vi "ADCS.UnlockECUSecurity.vi"(6 "Diagnostic Protocol":T3, 7 "Addon Name":string, 8 "error in (no error)":errorcluster, 9 "MasterKey":string, 10 "Security":T1={"Type"=enum."None", "Source DLL Path"=path "", "Target DLL Path"=path "", "Security Level"=1, "Static Master Key"="", "Max Key Length"=1, "Host IP Address"="", "ECU  Variant"=0, "Optional Parameter"=0}, 11 "diag ref in":T4={"Diag CAN Handle"=0, "Transport Protocol"=enum."ISO TP - Normal Mode", "Receive Address Extension"=0, "Transmit Address Extension"=0, "Receive CAN Id"=0, "Transmit CAN Id"=0, "Log Frames ?"=FALSE, "My TP Address"=0, "Other TP Address"=0, "T1"=0, "T2"=0, "T3"=0, "T4"=0, "Tx SN"=0, "Block Size"=0, "Rx SN"=0, "VW TP Initialized?"=FALSE, "Tx block no"=0, "baud rate"=0, "Interface"="", "Channel Diag CAN Handle"=0, "UDP Connection ID"=refnum, "TCP Connection ID"=refnum, "Target IP Addr"=0, "Source Address"=0, "Target Address"=0, "Send Header NACK?"=FALSE, "DLL Handle"=0, "NAD"=0, "Time Stamp read first"=0.0, "Time Stamp read last"=0.0, "Time Stamp write first"=0.0, "Time Stamp write last"=0.0, "Time Stamp write"=0.0, "Time Stamp read"=0.0, " I/O Mode"=0, "FD Baudrate"=0, "TX_DL"=8, "RX_DL"=8, "DoIP Protocol Version"=1, " Selected I/O Mode"=0, "TesterPresent Counter"=0, "TesterPresent Limit"=0, "TesterPresent Tick[ms]"=10, "TesterPresent RequireResponse?"=FALSE, "TesterPresent Stored Ref?"=FALSE, "TesterPresent Message"=[], "TesterPresent Task Handle"=0, "TesterPresent Semaphore"=refnum, "Response Plausibility Check"=1, "Default Version?"=TRUE, "Diagostic Globals"={"Timeout FC (Bs)"=250, "Timeout CF (Cr)"=250, "Timeout Diag Command"=1000, "Receive Block Size (BS)"=0, "Wait Time CF (STmin)"=5, "Max Waits (N_WFTmax)"=10, "Waits to Send (N_WAIT)"=0, "Time between Waits (TW)"=25, "Fill CAN Frames?"=TRUE, "Fill Byte"=255, "Invalid Response as Error?"=FALSE, "Max RspPending Count"=5, "VWTP Command Timeout"=50, "Transport Protocol"=enum."Diagnostics on IP", "Diag CAN Handle"=0, "DLL Handle"=0, "Timeout RspPending"=1000}, "Session-based Properties?"=FALSE, "NI-XNET IP Stack Reference"=0, "NI-XNET IP Stack TCP Reference"=-1, "NI-XNET IP Stack UDP Reference"=-1, "NI-XNET IP Stack Local Interface"="", "Functional CAN Id"=0, "Diag CAN Queue"=refnum, "Frame Fillling Mode"=0, "DoIP Acknowledge Mode"=0, "Message Buffer"=[]} {"Diagostic Globals"."Fill Byte" format="%x"; "TesterPresent Message" format="%.0x"; "Selected I/O Mode" items=["CAN", "CAN FD", "CAN FD+BRS", "ECU Determined"]; "DoIP Protocol Version" items=["2010"=1, "2012"=2]; "RX_DL" items=["8"=8, "12"=12, "16"=16, "20"=20, "24"=24, "32"=32, "48"=48, "64"=64]; "TX_DL" items=["8"=8, "12"=12, "16"=16, "20"=20, "24"=24, "32"=32, "48"=48, "64"=64]; "I/O Mode" items=["CAN", "CAN FD", "CAN FD+BRS", "Not yet determined"]}) -> (0 "error out":errorcluster, 1 "success?":bool, 3 "diag ref out":T4={"Diag CAN Handle"=0, "Transport Protocol"=enum."ISO TP - Normal Mode", "Receive Address Extension"=0, "Transmit Address Extension"=0, "Receive CAN Id"=0, "Transmit CAN Id"=0, "Log Frames ?"=FALSE, "My TP Address"=0, "Other TP Address"=0, "T1"=0, "T2"=0, "T3"=0, "T4"=0, "Tx SN"=0, "Block Size"=0, "Rx SN"=0, "VW TP Initialized?"=FALSE, "Tx block no"=0, "baud rate"=0, "Interface"="", "Channel Diag CAN Handle"=0, "UDP Connection ID"=refnum, "TCP Connection ID"=refnum, "Target IP Addr"=0, "Source Address"=0, "Target Address"=0, "Send Header NACK?"=FALSE, "DLL Handle"=0, "NAD"=0, "Time Stamp read first"=0.0, "Time Stamp read last"=0.0, "Time Stamp write first"=0.0, "Time Stamp write last"=0.0, "Time Stamp write"=0.0, "Time Stamp read"=0.0, " I/O Mode"=0, "FD Baudrate"=0, "TX_DL"=8, "RX_DL"=8, "DoIP Protocol Version"=1, " Selected I/O Mode"=0, "TesterPresent Counter"=0, "TesterPresent Limit"=0, "TesterPresent Tick[ms]"=10, "TesterPresent RequireResponse?"=FALSE, "TesterPresent Stored Ref?"=FALSE, "TesterPresent Message"=[], "TesterPresent Task Handle"=0, "TesterPresent Semaphore"=refnum, "Response Plausibility Check"=1, "Default Version?"=TRUE, "Diagostic Globals"={"Timeout FC (Bs)"=250, "Timeout CF (Cr)"=250, "Timeout Diag Command"=1000, "Receive Block Size (BS)"=0, "Wait Time CF (STmin)"=5, "Max Waits (N_WFTmax)"=10, "Waits to Send (N_WAIT)"=0, "Time between Waits (TW)"=25, "Fill CAN Frames?"=TRUE, "Fill Byte"=255, "Invalid Response as Error?"=FALSE, "Max RspPending Count"=5, "VWTP Command Timeout"=50, "Transport Protocol"=enum."Diagnostics on IP", "Diag CAN Handle"=0, "DLL Handle"=0, "Timeout RspPending"=1000}, "Session-based Properties?"=FALSE, "NI-XNET IP Stack Reference"=0, "NI-XNET IP Stack TCP Reference"=-1, "NI-XNET IP Stack UDP Reference"=-1, "NI-XNET IP Stack Local Interface"="", "Functional CAN Id"=0, "Diag CAN Queue"=refnum, "Frame Fillling Mode"=0, "DoIP Acknowledge Mode"=0, "Message Buffer"=[]} {"Diagostic Globals"."Fill Byte" format="%x"; "TesterPresent Message" format="%.0x"; "Selected I/O Mode" items=["CAN", "CAN FD", "CAN FD+BRS", "ECU Determined"]; "DoIP Protocol Version" items=["2010"=1, "2012"=2]; "RX_DL" items=["8"=8, "12"=12, "16"=16, "20"=20, "24"=24, "32"=32, "48"=48, "64"=64]; "TX_DL" items=["8"=8, "12"=12, "16"=16, "20"=20, "24"=24, "32"=32, "48"=48, "64"=64]; "I/O Mode" items=["CAN", "CAN FD", "CAN FD+BRS", "Not yet determined"]})   [LabVIEW 2024, in "Diagnostics Addon Engine.lvlib"]
uses:
  Diagnostics Addon Engine.lvlib
  <vilib>/Automotive Diagnostic Command Set/Diagnostic Transport.llb/Diag Reference.ctl
  <vilib>/Automotive Diagnostic Command Set/Diagnostic Transport.llb/Transport Protocol Selector.ctl
  <vilib>/Automotive Diagnostic Command Set/Diagnostic Transport.llb/DoIP Protocol Version.ctl
  <vilib>/Automotive Diagnostic Command Set/Diagnostic Transport.llb/Diag Globals.ctl
  Addon Shared/Types/Protocol.ctl
  Addon Shared/Types/Security.ctl
  Addon Shared/Types/Security.Type.ctl
  <vilib>/NI/STM/TCP/TCP Read Options.ctl
  <vilib>/NI/STM/TCP/Get Connection Reference (TCP).vi
  Support Libraries/GMLAN/_SubVIs/SecurityAccess_sendKey.vi
  <vilib>/NI/STM/TCP/Read Meta Data (TCP Ref).vi
  Support Libraries/GMLAN/_SubVIs/SecurityAccess_requestSeed.vi
  <vilib>/NI/STM/TCP/Read Meta Data (TCP Clst).vi
  <vilib>/Automotive Diagnostic Command Set/Diagnostic Transport.llb/Diagnostic Service.vi
  <vilib>/Automotive Diagnostic Command Set/Diagnostic Transport.llb/Apply Success Failure Error.vi
  <vilib>/Utility/error.llb/Error Cluster From Error Code.vi
  Support Libraries/GMLAN/GMLAN.lvlib
  <vilib>/NI/STM/NI STM.lvlib
  <vilib>/NI/NI VeriStand Addon Network Comm/Shared/NI VeriStand Addon Network Comm Shared.lvlib
  <vilib>/addons/Automotive Diagnostic Command Set/NI_Automotive Diagnostic Command Set.lvlib
  Addon Shared/Diagnostics Addon Shared.lvlib
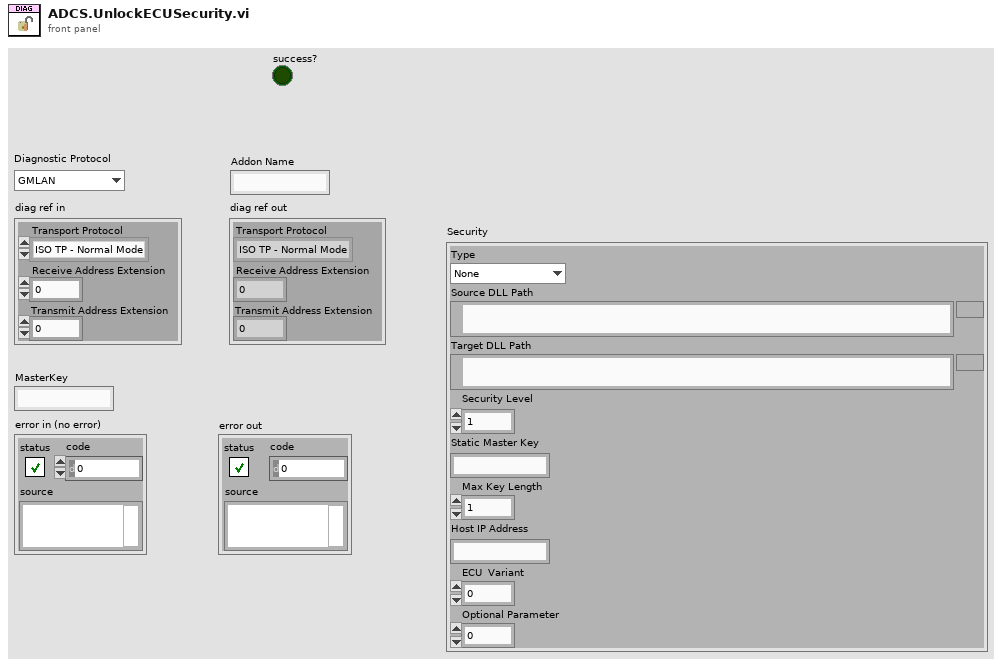
[diagram p1: front panel]
types:
  T1 = typedef "Diagnostics Addon Shared.lvlib/Security.ctl" = cluster{"Type":T2, "Source DLL Path":path, "Target DLL Path":path, "Security Level":u32, "Static Master Key":string, "Max Key Length":u32, "Host IP Address":string, "ECU  Variant":i8, "Optional Parameter":i8}
  T2 = typedef "Diagnostics Addon Shared.lvlib/Security.Type.ctl" = enum16{"None", "SeedKey DLL", "MasterKey (Channel)", "MasterKey (Static)", "SeedKey DLL (Windows)"}
  T3 = typedef "Diagnostics Addon Shared.lvlib/Protocol.ctl" = enum16{"GMLAN", "KWP-2000", "UDS", "User-Defined"}
  T4 = typedef "NI_Automotive Diagnostic Command Set.lvlib/Diag Reference.ctl" = cluster{"Diag CAN Handle":u32, "Transport Protocol":T5, "Receive Address Extension":u8, "Transmit Address Extension":u8, "Receive CAN Id":u32, "Transmit CAN Id":u32, "Log Frames ?":bool, "My TP Address":u8, "Other TP Address":u8, "T1":u16, "T2":u16, "T3":u16, "T4":u16, "Tx SN":u8, "Block Size":u8, "Rx SN":u8, "VW TP Initialized?":bool, "Tx block no":u8, "baud rate":u64, "Interface":string, "Channel Diag CAN Handle":u32, "UDP Connection ID":refnum<k16>, "TCP Connection ID":refnum<k5>, "Target IP Addr":u32, "Source Address":u16, "Target Address":u16, "Send Header NACK?":bool, "DLL Handle":u32, "NAD":u8, "Time Stamp read first":dbl, "Time Stamp read last":dbl, "Time Stamp write first":dbl, "Time Stamp write last":dbl, "Time Stamp write":dbl, "Time Stamp read":dbl, " I/O Mode":u32, "FD Baudrate":u64, "TX_DL":u16, "RX_DL":u16, "DoIP Protocol Version":T6, " Selected I/O Mode":u32, "TesterPresent Counter":u32, "TesterPresent Limit":u32, "TesterPresent Tick[ms]":i32, "TesterPresent RequireResponse?":bool, "TesterPresent Stored Ref?":bool, "TesterPresent Message":u8[], "TesterPresent Task Handle":i32, "TesterPresent Semaphore":T7, "Response Plausibility Check":u32, "Default Version?":bool, "Diagostic Globals":T8, "Session-based Properties?":bool, "NI-XNET IP Stack Reference":i64, "NI-XNET IP Stack TCP Reference":i64, "NI-XNET IP Stack UDP Reference":i64, "NI-XNET IP Stack Local Interface":string, "Functional CAN Id":u32, "Diag CAN Queue":refnum<queue>, "Frame Fillling Mode":u32, "DoIP Acknowledge Mode":u32, "Message Buffer":u8[]}
  T5 = typedef "NI_Automotive Diagnostic Command Set.lvlib/Transport Protocol Selector.ctl" = enum16{"ISO TP - Normal Mode", "ISO TP - Mixed Mode", "VW TP 2.0", "Diagnostics on IP", "ISO TP LIN"}
  T6 = typedef "NI_Automotive Diagnostic Command Set.lvlib/DoIP Protocol Version.ctl" = u8
  T7 = typedef "Semaphore RefNum" = refnum<k1>
  T8 = typedef "NI_Automotive Diagnostic Command Set.lvlib/Diag Globals.ctl" = cluster{"Timeout FC (Bs)":u32, "Timeout CF (Cr)":u32, "Timeout Diag Command":u32, "Receive Block Size (BS)":u8, "Wait Time CF (STmin)":u8, "Max Waits (N_WFTmax)":u8, "Waits to Send (N_WAIT)":i32, "Time between Waits (TW)":u32, "Fill CAN Frames?":bool, "Fill Byte":u32, "Invalid Response as Error?":bool, "Max RspPending Count":u32, "VWTP Command Timeout":u32, "Transport Protocol":T5, "Diag CAN Handle":u32, "DLL Handle":u32, "Timeout RspPending":u32}
  T9 = typedef "NI STM.lvlib/TCP Read Options.ctl" = cluster{"ignore timeout error":bool, "timeout ms (1000)":i32}
  T10 = typedef "NI STM.lvlib/TCP Connection Info.ctl" = cluster{"connection ID":refnum<k5>, "meta data":T11[]}
  T11 = typedef "NI STM.lvlib/MetaDataElement.ctl" = string
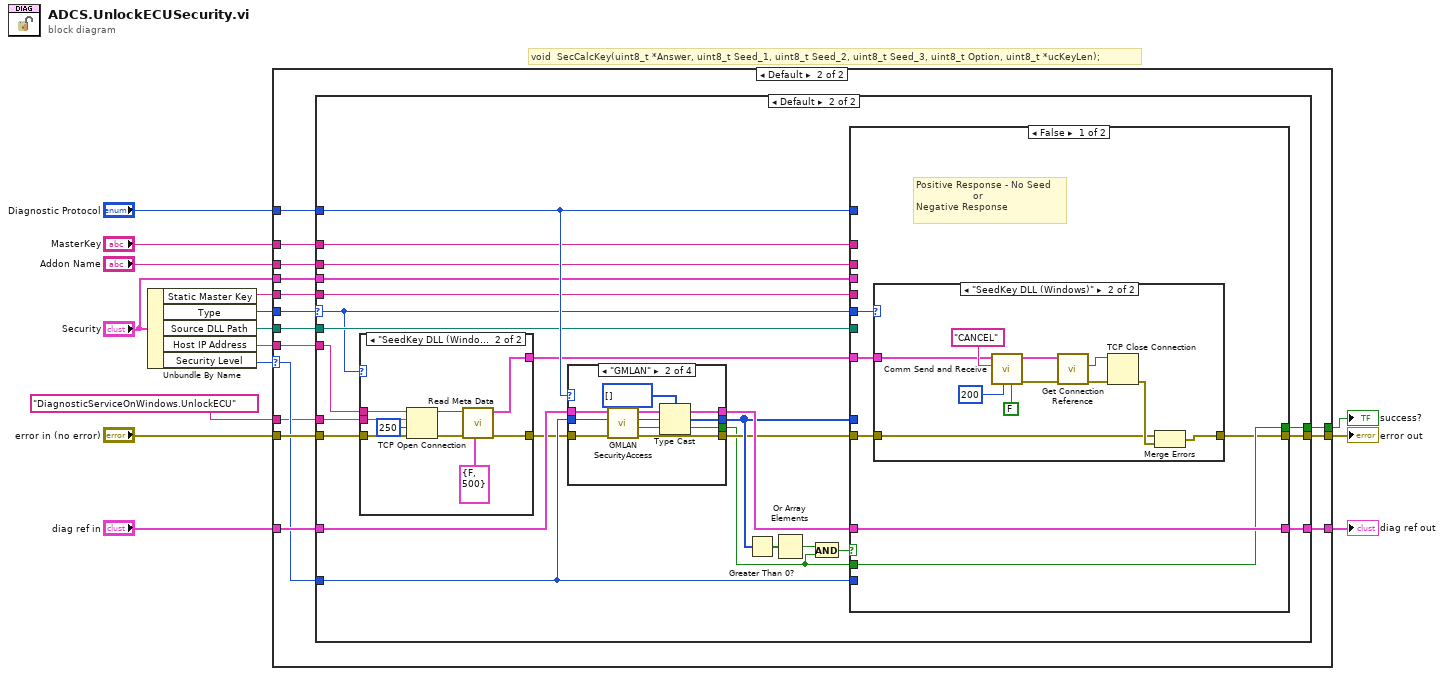
[diagram p0: block diagram]
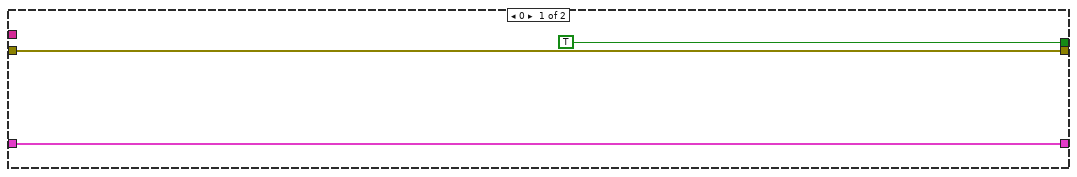
[diagram p2: hidden frame]
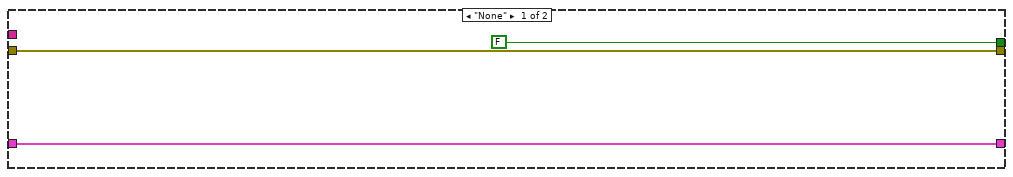
[diagram p3: hidden frame]
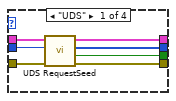
[diagram p5: hidden frame]
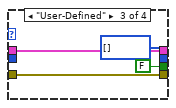
[diagram p6: hidden frame]
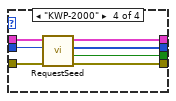
[diagram p7: hidden frame]
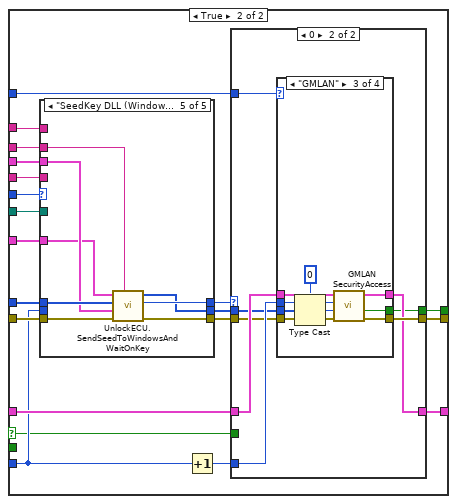
[diagram p9: hidden frame]
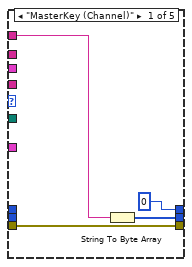
[diagram p10: hidden frame]
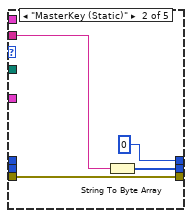
[diagram p11: hidden frame]
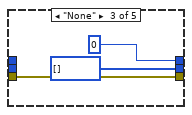
[diagram p12: hidden frame]
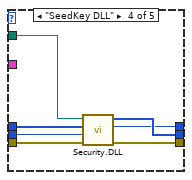
[diagram p13: hidden frame]
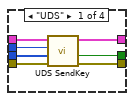
[diagram p15: hidden frame]
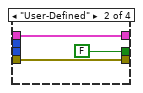
[diagram p16: hidden frame]
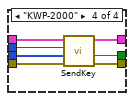
[diagram p17: hidden frame]
diagram:
  # "void  SecCalcKey(uint8_t *Answer, uint8_t Seed_1, uint8_t Seed_2, uint8_t Seed_3, uint8_t Option, uint8_t *ucKeyLen);"
  n1 = Unbundle By Name("Security") -> ("Static Master Key"=w5:string, "Type"=w7:T2, "Source DLL Path"=w10:path, "Host IP Address"=w1:string, "Security Level"=w9:u32)
  n2 = case shown="Default" w9 {
    selector: w9 -> [_ w27]
    tunnel: "diag ref in" -> [w18 w33]
    tunnel: [w18 w32] -> w14
    tunnel: "Diagnostic Protocol" -> [_ w31]
    tunnel: "error in (no error)" -> [w17 w30]
    tunnel: [w17 w29] -> w11
    tunnel: w10 -> [_ w28]
    tunnel: [TRUE ("success?") w26] -> w8
    tunnel: w7 -> [_ w25]
    tunnel: "MasterKey" -> [_ w24]
    tunnel: w5 -> [_ w23]
    tunnel: "Security" -> [_ w22]
    tunnel: "Addon Name" -> [_ w21]
    tunnel: "DiagnosticServiceOnWindows.UnlockECU" ("Host IP Address") -> [_ w20]
    tunnel: w1 -> [_ w19]
    frame 0 {
    }
    frame Default {
      n3 = case shown="Default" w25 {
        selector: w25 -> [_ w40]
        tunnel: w33 -> [w36 w60]
        tunnel: [w36 w59] -> w32
        tunnel: w31 -> [_ w55]
        tunnel: w30 -> [w35 w42]
        tunnel: [w35 w51] -> w29
        tunnel: w28 -> [_ w50]
        tunnel: w27 -> [_ w49]
        tunnel: [FALSE ("success?") w47] -> w26
        tunnel: w24 -> [_ w46]
        tunnel: w23 -> [_ w45]
        tunnel: w22 -> [_ w44]
        tunnel: w21 -> [_ w43]
        tunnel: w20 -> [_ w39]
        tunnel: w19 -> [_ w38]
        frame "None" {
        }
        frame Default {
          n4 = case shown="\"SeedKey DLL (Windows)\"" w40 {
            tunnel: w42 -> [w61 w66]
            tunnel: [w61 w65] -> w41
            tunnel: w39 -> [_ w64]
            tunnel: w38 -> [_ w63]
            tunnel: [_ w62] -> w37
            frame Default {
            }
            frame "SeedKey DLL (Windows)" {
              n5 = TCP Open Connection(address=w63, remote port or service name=w64, timeout ms (60000)=250, error in (no error)=w66) -> (connection ID=w70:refnum<k5>, error out=w69:errorcluster)  [unwired: 1 in]
              n6 = call-poly <vilib>:"Read Meta Data.vi"("options"=T9 {"ignore timeout error"=FALSE, "timeout ms (1000)"=500}, "error in"=w69, "connection ID"=w70) -> ("error out"=w65:errorcluster, "connection info out"=w62:T10)  [unwired: 6 in, 1 out]
            }
          }
          n7 = case shown="\"GMLAN\"" w55 {
            tunnel: w41 -> [w74 w84 w90 w97]
            tunnel: w60 -> [w75 w86 w89 w96]
            tunnel: [w71 w81 w89 w95] -> w54
            tunnel: w49 -> [w76 w85 _ w94]
            tunnel: [w73 w83 w90 w93] -> w52
            tunnel: [w72 w78 u8[] [] ("seed out") w92] -> w53
            tunnel: [w77 w82 FALSE ("success?") w91] -> w48
            frame "UDS" {
              n8 = call <vilib>:"UDS RequestSeed.vi"("error in (no error)"=w74, "access mode"=w76, "diag ref in"=w75) -> ("error out"=w73:errorcluster, "success?"=w77:bool, "seed out"=w72:u8[], "diag ref out"=w71:T4)  [unwired: 5 in]
            }
            frame "GMLAN" {
              n9 = call-poly "GMLAN SecurityAccess.vi"("error in (no error)"=w84, "subFunction"=w85, "diag ref in"=w86) -> ("error out"=w83:errorcluster, "success?"=w82:bool, "SecuritySeed"=w80:u16, "diag ref out"=w81:T4)  [unwired: 5 in]
              n10 = Type Cast(type=u8[] [] ("seed out"), x=w80) -> (*(type *) &x=w78:u8[])
            }
            frame "User-Defined" {
            }
            frame "KWP-2000" {
              n11 = call <vilib>:"RequestSeed.vi"("error in (no error)"=w97, "access mode"=w94, "diag ref in"=w96) -> ("error out"=w93:errorcluster, "success?"=w91:bool, "seed out"=w92:u8[], "diag ref out"=w95:T4)  [unwired: 5 in]
            }
          }
          n12 = Greater Than 0?(x=w53) -> (x > 0?=w58:bool[])
          n13 = Or Array Elements(Boolean array=w58) -> (logical OR=w56:bool)
          n14 = And(x=w56, y=w48) -> (x .and. y?=w57:bool)
          n15 = case shown="False" w57 {
            selector: w57 -> [_ w123]
            tunnel: [w99 w135] -> w51
            tunnel: w50 -> [_ w129]
            tunnel: w54 -> [w103 w134]
            tunnel: w53 -> [_ w130]
            tunnel: w52 -> [w98 w131]
            tunnel: [w103 w133] -> w59
            tunnel: w49 -> [_ w125]
            tunnel: w55 -> [_ w132]
            tunnel: [w102 w122] -> w47
            tunnel: w48 -> [w102 _]
            tunnel: w40 -> [w100 w121]
            tunnel: w46 -> [_ w120]
            tunnel: w45 -> [_ w119]
            tunnel: w44 -> [_ w118]
            tunnel: w43 -> [_ w117]
            tunnel: w37 -> [w101 w116]
            frame False {
              # "Positive Response - No Seed\n                   or\nNegative Response"
              n16 = case shown="\"SeedKey DLL (Windows)\"" w100 {
                tunnel: w98 -> [w104 w111]
                tunnel: w101 -> [_ w107]
                tunnel: [w104 w112] -> w99
                frame Default {
                }
                frame "SeedKey DLL (Windows)" {
                  n17 = call <vilib>:"Comm Send and Receive.vi"("Resp Required?"=FALSE, "Timeout (ms)"=u32 200, "Name"="CANCEL", "connection info"=w107) -> ("error out"=w105:errorcluster, "connection info"=w106:T10)  [unwired: 4 in, 2 out]
                  n18 = call-poly <vilib>:"Get Connection Reference.vi"("error in"=w105, "connection info in"=w106) -> ("error out"=w114:errorcluster, "connection ID out"=w115:refnum<k5>)  [unwired: 7 in, 1 out]
                  n19 = TCP Close Connection(connection ID=w115, error in (no error)=w114) -> (error out=w113:errorcluster)  [unwired: 1 in, 1 out]
                  n20 = Merge Errors(w111, w113) -> (w112:errorcluster)
                }
              }
            }
            frame True {
              n21 = case shown="\"SeedKey DLL (Windows)\"" w121 {
                tunnel: w131 -> [w138 w142 w146 w153 w161]
                tunnel: w130 -> [_ _ _ w152 w156]
                tunnel: w129 -> [_ _ _ w151 _]
                tunnel: [w139 w143 u8[] [] ("unsigned byte array") w150 w158] -> w128
                tunnel: [u8 0 ("lockstatus") u8 0 ("lockstatus") u8 0 ("lockstatus") w149 w160] -> w127
                tunnel: [w138 w142 w146 w148 w159] -> w126
                tunnel: w125 -> [_ _ _ w147 _]
                tunnel: w120 -> [w136 _ _ _ _]
                tunnel: w119 -> [_ w140 _ _ _]
                tunnel: w118 -> [_ _ _ _ w155]
                tunnel: w117 -> [_ _ _ _ w157]
                tunnel: w116 -> [_ _ _ _ w154]
                frame "MasterKey (Channel)" {
                  n22 = String To Byte Array(string=w136) -> (unsigned byte array=w139:u8[])
                }
                frame "MasterKey (Static)" {
                  n23 = String To Byte Array(string=w140) -> (unsigned byte array=w143:u8[])
                }
                frame "None" {
                }
                frame "SeedKey DLL" {
                  n24 = call "Security.DLL.vi"("error in (no error)"=w153, "Option"=w147, "Seed"=w152, "path in"=w151) -> ("error out"=w148:errorcluster, "lockstatus"=w149:u8, "unsigned byte array"=w150:u8[])  [unwired: 5 in]
                }
                frame "SeedKey DLL (Windows)" {
                  n25 = call "UnlockECU.SendSeedToWindowsAndWaitOnKey.vi"("Addon Name"=w157, "error in (no error)"=w161, "Security"=w155, "Seed"=w156, "TCP Info"=w154) -> ("error out"=w159:errorcluster, "Error code"=w160:i32, "Key"=w158:u8[])  [unwired: 4 in]
                }
              }
              n26 = Increment(x=w125) -> (x+1=w124:u32)
              n27 = case shown="0" w127 {
                tunnel: [w164 w172] -> w135
                tunnel: w134 -> [w163 w171]
                tunnel: [w163 w170] -> w133
                tunnel: w124 -> [_ w169]
                tunnel: w132 -> [_ w168]
                tunnel: w126 -> [w164 w167]
                tunnel: w128 -> [_ w166]
                tunnel: [w162 w165] -> w122
                tunnel: w123 -> [w162 _]
                frame Default {
                }
                frame 0 {
                  n28 = case shown="\"GMLAN\"" w168 {
                    tunnel: [w177 w182 w188 w198] -> w172
                    tunnel: w171 -> [w179 w181 w190 w197]
                    tunnel: w167 -> [w176 w182 w189 w196]
                    tunnel: [w178 w181 w187 w195] -> w170
                    tunnel: w169 -> [w174 _ w191 w194]
                    tunnel: w166 -> [w175 _ w186 w193]
                    tunnel: [w173 FALSE ("success?") w183 w192] -> w165
                    frame "UDS" {
                      n29 = call <vilib>:"UDS SendKey.vi"("error in (no error)"=w176, "key in"=w175, "access mode"=w174, "diag ref in"=w179) -> ("error out"=w177:errorcluster, "success?"=w173:bool, "diag ref out"=w178:T4)  [unwired: 5 in]
                    }
                    frame "User-Defined" {
                    }
                    frame "GMLAN" {
                      n30 = Type Cast(type=u16 0 ("SecuritySeed"), x=w186) -> (*(type *) &x=w185:u16)
                      n31 = call-poly "GMLAN SecurityAccess.vi"("error in (no error)"=w189, "SecuritySeed"=w185, "subFunction"=w191, "diag ref in"=w190) -> ("error out"=w188:errorcluster, "success?"=w183:bool, "diag ref out"=w187:T4)  [unwired: 5 in]
                    }
                    frame "KWP-2000" {
                      n32 = call <vilib>:"SendKey.vi"("error in (no error)"=w196, "key in"=w193, "access mode"=w194, "diag ref in"=w197) -> ("error out"=w198:errorcluster, "success?"=w192:bool, "diag ref out"=w195:T4)  [unwired: 5 in]
                    }
                  }
                }
              }
            }
          }
        }
      }
    }
  }
  "error out" <- w11
  "diag ref out" <- w14
  "success?" <- w8
